vi "Generate Parameters Typedef Name.vi"(8 "error in":errorcluster, 10 "Parameter Mode":T1, 11 "VI Name":string) -> (0 "error out":errorcluster, 3 "Type Definition Name":string)   [LabVIEW 2026]
doc: "This VI generates the input/output parameter type definifion name from a VIs name."
uses:
  Type Definitions/Parameter Mode--enum.ctl
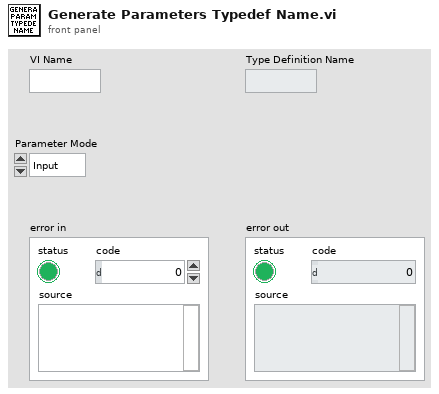
[diagram p1: front panel]
types:
  T1 = typedef "Parameter Mode--enum.ctl" = enum16{"Input", "Output"}
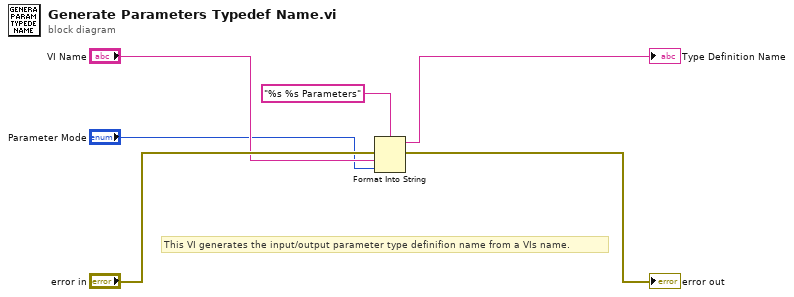
[diagram p0: block diagram]
diagram:
  # "This VI generates the input/output parameter type definifion name from a VIs name."
  n1 = Format Into String(format string="%s %s Parameters", error in="error in", "VI Name", "Parameter Mode") -> (resulting string=→"Type Definition Name":string, error out=→"error out":errorcluster)  [unwired: 1 in]
